vi "Init.vi"(8 "error in (no error)":errorcluster caption="에러 입력(에러 없음)", 9 "Sad Queue":refnum<queue>, 10 "Queue Ref":T1, 11 "Instrument Manager 입력":refnum<class "Instrument Manager.lvclass">) -> (0 "error out":errorcluster caption="에러 출력", 3 "Instrument Manager 출력":refnum<class "Instrument Manager.lvclass">)   [LabVIEW 2023, in "Instrument Manager.lvclass"]
uses:
  Instrument Manager.lvclass
  Instrument Manager.lvclass/Instrument Manager.ctl
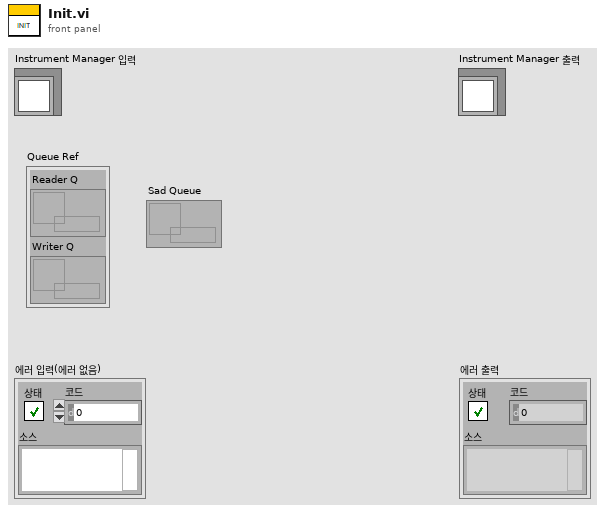
[diagram p1: front panel]
types:
  T1 = cluster{"Reader Q":refnum<queue>, "Writer Q":refnum<queue>}
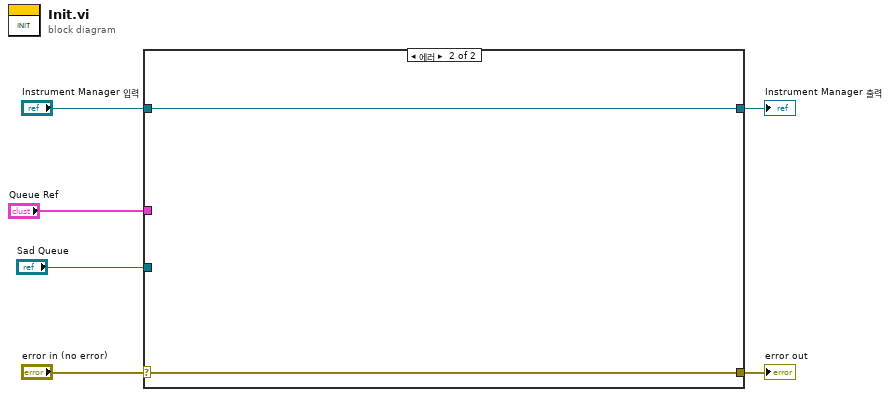
[diagram p0: block diagram]
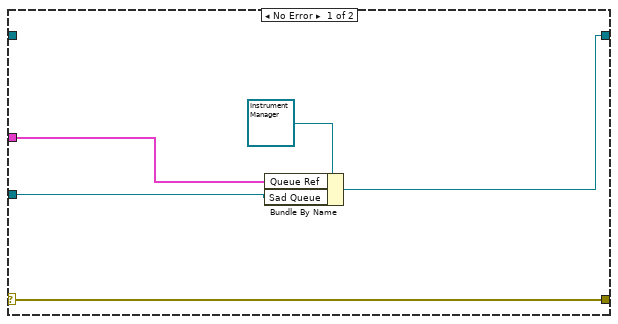
[diagram p2: hidden frame]
diagram:
  n1 = case shown="에러" "error in (no error)" {
    selector: "error in (no error)" -> [w11 w13]
    tunnel: [w11 w13] -> w5
    tunnel: [w7 w12] -> w3
    tunnel: "Instrument Manager 입력" -> [_ w12]
    tunnel: "Queue Ref" -> [w9 _]
    tunnel: "Sad Queue" -> [w8 _]
    frame No Error {
      n2 = Bundle By Name(cluster=refnum<class "Instrument Manager.lvclass"> refnum ("Instrument Manager.lvclass"), "Queue Ref"=w9, "Sad Queue"=w8) -> (w7:refnum<class "Instrument Manager.lvclass">)
    }
    frame Error {
    }
  }
  "error out" <- w5
  "Instrument Manager 출력" <- w3
